vi "Init_Reg.vi"(0 "connection ID in":refnum<k5>, 2 "EVT_TAIL":i32=300, 3 "TRIG_DT":i32=500, 4 "EVT_LEN":i32=400, 5 "BL_LEN":i32=50, 6 "error in":errorcluster, 7 "TRIG_TH":i32=200) -> (1 "error out":errorcluster)   [LabVIEW 2014]
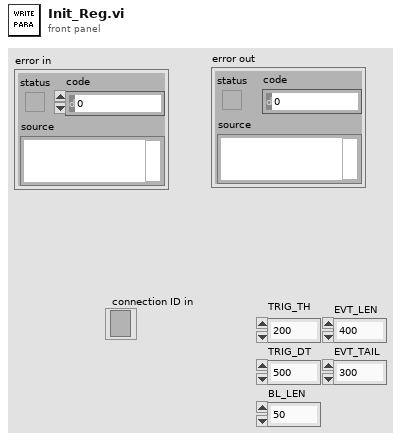
[diagram p1: front panel]
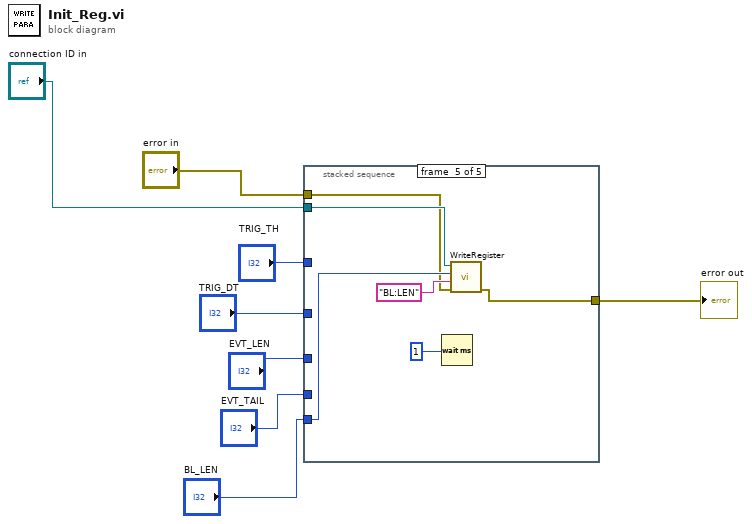
[diagram p0: block diagram]
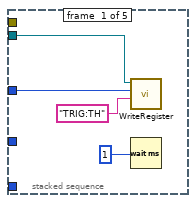
[diagram p2: hidden frame]
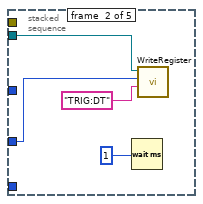
[diagram p3: hidden frame]
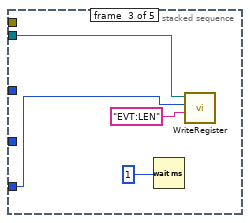
[diagram p4: hidden frame]
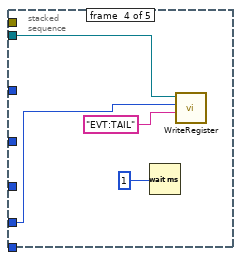
[diagram p5: hidden frame]
diagram:
  n1 = stacked-sequence {
    tunnel: "TRIG_TH" -> [w10 _ _ _ _]
    tunnel: "connection ID in" -> [w9 w13 w18 w22 w28]
    tunnel: "TRIG_DT" -> [_ w14 _ _ _]
    tunnel: "EVT_LEN" -> [_ _ w17 _ _]
    tunnel: "EVT_TAIL" -> [_ _ _ w23 _]
    tunnel: "BL_LEN" -> [_ _ _ _ w29]
    tunnel: [_ _ _ _ w26] -> w2
    tunnel: "error in" -> [_ _ _ _ w25]
    frame #0 {
      n2 = call "WriteRegister.vi"("string in"="TRIG:TH", "value in"=w10, "connection ID in"=w9) -> ()  [unwired: 5 in, 2 out]
      n3 = Wait (ms)(milliseconds to wait=1 ("Value")) -> ()  [unwired: 1 out]
    }
    frame #1 {
      n4 = Wait (ms)(milliseconds to wait=1 ("Value")) -> ()  [unwired: 1 out]
      n5 = call "WriteRegister.vi"("string in"="TRIG:DT", "value in"=w14, "connection ID in"=w13) -> ()  [unwired: 5 in, 2 out]
    }
    frame #2 {
      n6 = Wait (ms)(milliseconds to wait=1 ("Value")) -> ()  [unwired: 1 out]
      n7 = call "WriteRegister.vi"("string in"="EVT:LEN", "value in"=w17, "connection ID in"=w18) -> ()  [unwired: 5 in, 2 out]
    }
    frame #3 {
      n8 = Wait (ms)(milliseconds to wait=1 ("Value")) -> ()  [unwired: 1 out]
      n9 = call "WriteRegister.vi"("string in"="EVT:TAIL", "value in"=w23, "connection ID in"=w22) -> ()  [unwired: 5 in, 2 out]
    }
    frame #4 {
      n10 = Wait (ms)(milliseconds to wait=1 ("Value")) -> ()  [unwired: 1 out]
      n11 = call "WriteRegister.vi"("error in"=w25, "string in"="BL:LEN", "value in"=w29, "connection ID in"=w28) -> ("error out"=w26:errorcluster)  [unwired: 4 in, 1 out]
    }
  }
  "error out" <- w2
